vi "0Ludwieg_automation.vi"() -> ()   [LabVIEW 2025]
uses:
  State.ctl
  <vilib>/DAQmx/write.llb/DAQmx Write (Digital Bool 1Line 1Point).vi
  <vilib>/DAQmx/read.llb/DAQmx Read (Analog 2D DBL NChan NSamp).vi
  <vilib>/Analysis/baseanly.llb/Mean (DBL).vi
  <vilib>/DAQmx/write.llb/DAQmx Write (Analog 2D DBL NChan NSamp).vi
  <vilib>/DAQmx/write.llb/DAQmx Write (Digital 1D U32 1Chan NSamp).vi
  <vilib>/DAQmx/write.llb/DAQmx Write (Analog 1D DBL NChan 1Samp).vi
  <vilib>/DAQmx/create/channels.llb/DAQmx Create Channel (DO-Digital Output).vi
  <vilib>/DAQmx/create/channels.llb/DAQmx Create Channel (AI-Voltage-Basic).vi
  <vilib>/DAQmx/configure/timing.llb/DAQmx Timing (Sample Clock).vi
  <vilib>/DAQmx/configure/trigger.llb/DAQmx Start Trigger (Digital Edge).vi
  <vilib>/DAQmx/create/channels.llb/DAQmx Create Channel (AO-Voltage-Basic).vi
  <vilib>/DAQmx/miscellaneous.llb/DAQmx Fill In Error Info.vi
  <vilib>/Analysis/NI_AALBase.lvlib
  <resource>/objmgr/daqmx.rc
panel:
  out "Write_OK":bool
  in  "Done?":bool
  in  "Write?":bool
  in  "Start_path":path=path "C:/Users/IITH/Desktop"
  out "Saved_file_path":path
  out "Last_run?":bool
  in  "Next_run?":bool
  out "Timing_OK":bool
  out "Timing_msg":string
  out "gate_start_ms":dbl
  in  "trigger_gap_ms":dbl=-1.0
  in  "Cam_gate_len_ms":dbl=40.0
  in  "pre_flow_ms":dbl=15.0
  in  "flow_lag_ms":dbl=30.0
  in  "valve_delay":dbl=100.0
  in  "Valve_pulse_ms":dbl=30.0
  out "Camera_delay":dbl=50.0
  in  "Camera_pulse_ms":dbl=50.0
  out "Pulse_length_ms":dbl=500.0
  in  "AI_Start_delay_ms":dbl=115.0
  in  "AI_Capture_ms":dbl=40.0
  out "Run_count":i32
  in  "N_runs":i32=1 min=1 max=10 step=1
  out "Iteration":i32
  out "Current_state":T1
  in  "AI_data_record_Ch":tag="Dev1/ai0:3"
  out "Actual_AI_Rate":dbl
  in  "Frequency (Hz)":dbl=300000.0 format="%0.2f"
  in  "Abort":bool
  in  "Force_stop":bool
  in  "Vac_pump_DO_Ch":tag="Dev1/port1/line1"
  in  "Fire_AO_Ch":tag="Dev1/ao0:1"
  in  "AI_input_config":i32(ring)=10106 items=["Default"=-1, "RSE"=10083, "NRSE"=10078, "Differential"=10106, "Pseudodifferential"=12529]
  in  "Global_driver_rate":dbl=1000.0 format="%0.2f"
  in  "Exhaust_SSR_Ch":tag="Dev2/ao1"
  in  "Inlet_SSR_Ch":tag="Dev2/ao0"
  out "Vac_Pump":bool
  out "Abort_state":bool
  out "P_vac_Pa":dbl
  out "P_driver_Pa":dbl
  out "Fill_cutoff_Pa":dbl format="%.4f"
  out "Vac_cutoff_Pa":dbl format="%.4f"
  in  "Driver_units":enum16{"psi", "bar", "kPa", "Pa"}(ring)=enum."bar"
  in  "Vacuum_units":enum16{"psi", "bar", "kPa", "Pa"}(ring)=enum."Pa"
  in  "P_driver_target":dbl=10.0
  in  "P_vac_target":dbl=6.0
  in  "Vac_pressure_Ch":tag="Dev2/ai0"
  in  "Driver_pressure_Ch":tag="Dev2/ai1"
  out "Driver_gauge_%":dbl(knob) scale=0.0..130.0
  out "Vac_gauge_%":dbl(knob)
  out "Sensor_fault":bool
  out "Control_pressures":dbl[][](graph)
  out "6374_data_output":dbl[][](graph)
  out "Trigger_pulse_waveform":dbl[][](graph)=[[0.0, 0.0, 0.0, 0.0, 0.0, 0.0, 0.0, 0.0, 0.0, 0.0, 0.0, 0.0, 0.0, 0.0, 0.0, 0.0, 0.0, 0.0, 0.0, 0.0, 0.0, 0.0, 0.0, 0.0, 0.0, 0.0, 0.0, 0.0, 0.0, 0.0, 0.0, 0.0, 0.0, 0.0, 0.0, 0.0, 0.0, 0.0, 0.0, 0.0, 0.0, 0.0, 0.0, 0.0, 0.0, 0.0, 0.0, 0.0, 0.0, 0.0, 0.0, 0.0, 0.0, 0.0, 0.0, 0.0, 0.0, 0.0, 0.0, 0.0, 0.0, 0.0, 0.0, 0.0, 0.0, 0.0, 0.0, 0.0, 0.0, 0.0, 0.0, 0.0, 0.0, 0.0, 0.0, 0.0, 0.0, 0.0, 0.0, 0.0, 0.0, 0.0, 0.0, 0.0, 0.0, 0.0, 0.0, 0.0, 0.0, 0.0, 0.0, 0.0, 0.0, 0.0, 0.0, 0.0, 0.0, 0.0, 0.0, 0.0, 4.9, 4.9, 4.9, 4.9, 4.9, 4.9, 4.9, 4.9, 4.9, 4.9, 4.9, 4.9, 4.9, 4.9, 4.9, 4.9, 4.9, 4.9, 4.9, 4.9, 4.9, 4.9, 4.9, 4.9, 4.9, 4.9, 4.9, 4.9, 4.9, 4.9, 4.9, 4.9, 4.9, 4.9, 4.9, 4.9, 4.9, 4.9, 4.9, 4.9, 4.9, 4.9, 4.9, 4.9, 4.9, 4.9, 4.9, 4.9, 4.9, 4.9, 0.0, 0.0, 0.0, 0.0, 0.0, 0.0, 0.0, 0.0, 0.0, 0.0, 0.0, 0.0, 0.0, 0.0, 0.0, 0.0, 0.0, 0.0, 0.0, 0.0, 0.0, 0.0, 0.0, 0.0, 0.0, 0.0, 0.0, 0.0, 0.0, 0.0, 0.0, 0.0, 0.0, 0.0, 0.0, 0.0, 0.0, 0.0, 0.0, 0.0, 0.0, 0.0, 0.0, 0.0, 0.0, 0.0, 0.0, 0.0, 0.0, 0.0, 0.0, 0.0, 0.0, 0.0, 0.0, 0.0, 0.0, 0.0, 0.0, 0.0, 0.0, 0.0, 0.0, 0.0, 0.0, 0.0, 0.0, 0.0, 0.0, 0.0, 0.0, 0.0, 0.0, 0.0, 0.0, 0.0, 0.0, 0.0, 0.0, 0.0, 0.0, 0.0, 0.0, 0.0, 0.0, 0.0, 0.0, 0.0, 0.0, 0.0, 0.0, 0.0, 0.0, 0.0, 0.0, 0.0, 0.0, 0.0, 0.0, 0.0, 0.0, 0.0, 0.0, 0.0, 0.0, 0.0, 0.0, 0.0, 0.0, 0.0, 0.0, 0.0, 0.0, 0.0, 0.0, 0.0, 0.0, 0.0, 0.0, 0.0, 0.0, 0.0, 0.0, 0.0, 0.0, 0.0, 0.0, 0.0, 0.0, 0.0, 0.0, 0.0, 0.0, 0.0, 0.0, 0.0, 0.0, 0.0, 0.0, 0.0, 0.0, 0.0, 0.0, 0.0, 0.0, 0.0, 0.0, 0.0, 0.0, 0.0, 0.0, 0.0, 0.0, 0.0, 0.0, 0.0, 0.0, 0.0, 0.0, 0.0, 0.0, 0.0, 0.0, 0.0, 0.0, 0.0, 0.0, 0.0, 0.0, 0.0, 0.0, 0.0, 0.0, 0.0, 0.0, 0.0, 0.0, 0.0, 0.0, 0.0, 0.0, 0.0, 0.0, 0.0, 0.0, 0.0, 0.0, 0.0, 0.0, 0.0, 0.0, 0.0, 0.0, 0.0, 0.0, 0.0, 0.0, 0.0, 0.0, 0.0, 0.0, 0.0, 0.0, 0.0, 0.0, 0.0, 0.0, 0.0, 0.0, 0.0, 0.0, 0.0, 0.0, 0.0, 0.0, 0.0, 0.0, 0.0, 0.0, 0.0, 0.0, 0.0, 0.0, 0.0, 0.0, 0.0, 0.0, 0.0, 0.0, 0.0, 0.0, 0.0, 0.0, 0.0, 0.0, 0.0, 0.0, 0.0, 0.0, 0.0, 0.0, 0.0, 0.0, 0.0, 0.0, 0.0, 0.0, 0.0, 0.0, 0.0, 0.0, 0.0, 0.0, 0.0, 0.0, 0.0, 0.0, 0.0, 0.0, 0.0, 0.0, 0.0, 0.0, 0.0, 0.0, 0.0, 0.0, 0.0, 0.0, 0.0, 0.0, 0.0, 0.0, 0.0, 0.0, 0.0, 0.0, 0.0, 0.0, 0.0, 0.0, 0.0, 0.0, 0.0, 0.0, 0.0, 0.0, 0.0, 0.0, 0.0, 0.0, 0.0, 0.0, 0.0, 0.0, 0.0, 0.0, 0.0, 0.0, 0.0, 0.0, 0.0, 0.0, 0.0, 0.0, 0.0, 0.0, 0.0, 0.0, 0.0, 0.0, 0.0, 0.0, 0.0, 0.0, 0.0, 0.0, 0.0, 0.0, 0.0, 0.0, 0.0, 0.0, 0.0, 0.0, 0.0, 0.0, 0.0, 0.0, 0.0, 0.0, 0.0, 0.0, 0.0, 0.0, 0.0, 0.0, 0.0, 0.0, 0.0, 0.0, 0.0, 0.0, 0.0, 0.0, 0.0, 0.0, 0.0, 0.0, 0.0, 0.0, 0.0, 0.0, 0.0, 0.0, 0.0, 0.0, 0.0, 0.0, 0.0, 0.0, 0.0, 0.0, 0.0, 0.0, 0.0, 0.0, 0.0, 0.0, 0.0, 0.0, 0.0, 0.0, 0.0, 0.0, 0.0, 0.0, 0.0, 0.0, 0.0, 0.0, 0.0, 0.0, 0.0, 0.0, 0.0, 0.0, 0.0, 0.0, 0.0, 0.0, 0.0, 0.0, 0.0, 0.0, 0.0, 0.0, 0.0, 0.0, 0.0, 0.0, 0.0, 0.0, 0.0, 0.0, 0.0, 0.0, 0.0, 0.0, 0.0, 0.0, 0.0, 0.0, 0.0, 0.0, 0.0, 0.0, 0.0, 0.0, 0.0, 0.0, 0.0, 0.0, 0.0, 0.0, 0.0, 0.0, 0.0, 0.0, 0.0, 0.0, 0.0, 0.0, 0.0, 0.0, 0.0, 0.0, 0.0, 0.0, 0.0, 0.0, 0.0, 0.0, 0.0, 0.0, 0.0, 0.0, 0.0, 0.0, 0.0, 0.0, 0.0, 0.0, 0.0, 0.0, 0.0, 0.0, 0.0, 0.0, 0.0, 0.0, 0.0, 0.0, 0.0, 0.0, 0.0, 0.0, 0.0, 0.0, 0.0, 0.0, 0.0, 0.0, 0.0, 0.0, 0.0, 0.0, 0.0, 0.0, 0.0, 0.0, 0.0, 0.0, 0.0, 0.0, 0.0, 0.0, 0.0, 0.0, 0.0, 0.0, 0.0, 0.0, 0.0, 0.0, 0.0, 0.0, 0.0, 0.0, 0.0, 0.0, 0.0, 0.0, 0.0, 0.0, 0.0, 0.0, 0.0, 0.0, 0.0, 0.0, 0.0, 0.0, 0.0, 0.0, 0.0, 0.0, 0.0, 0.0, 0.0, 0.0, 0.0, 0.0, 0.0, 0.0, 0.0, 0.0, 0.0, 0.0, 0.0, 0.0, 0.0, 0.0, 0.0, 0.0, 0.0, 0.0, 0.0, 0.0, 0.0, 0.0, 0.0, 0.0, 0.0, 0.0, 0.0, 0.0, 0.0, 0.0, 0.0, 0.0, 0.0, 0.0, 0.0, 0.0, 0.0, 0.0, 0.0, 0.0, 0.0, 0.0, 0.0, 0.0, 0.0, 0.0, 0.0, 0.0, 0.0, 0.0, 0.0, 0.0, 0.0, 0.0, 0.0, 0.0, 0.0, 0.0, 0.0, 0.0, 0.0, 0.0, 0.0, 0.0, 0.0, 0.0, 0.0, 0.0, 0.0, 0.0, 0.0, 0.0, 0.0, 0.0, 0.0, 0.0, 0.0, 0.0, 0.0, 0.0, 0.0, 0.0, 0.0, 0.0, 0.0, 0.0, 0.0, 0.0, 0.0, 0.0, 0.0, 0.0, 0.0, 0.0, 0.0, 0.0, 0.0, 0.0, 0.0, 0.0, 0.0, 0.0, 0.0, 0.0, 0.0, 0.0, 0.0, 0.0, 0.0, 0.0, 0.0, 0.0, 0.0, 0.0, 0.0, 0.0, 0.0, 0.0, 0.0, 0.0, 0.0, 0.0, 0.0, 0.0, 0.0, 0.0, 0.0, 0.0, 0.0, 0.0, 0.0, 0.0, 0.0, 0.0, 0.0, 0.0, 0.0, 0.0, 0.0, 0.0, 0.0, 0.0, 0.0, 0.0, 0.0, 0.0, 0.0, 0.0, 0.0, 0.0, 0.0, 0.0, 0.0, 0.0, 0.0, 0.0, 0.0, 0.0, 0.0, 0.0, 0.0, 0.0, 0.0, 0.0, 0.0, 0.0, 0.0, 0.0, 0.0, 0.0, 0.0, 0.0, 0.0, 0.0, 0.0, 0.0, 0.0, 0.0, 0.0, 0.0, 0.0, 0.0, 0.0, 0.0, 0.0, 0.0, 0.0, 0.0, 0.0, 0.0, 0.0, 0.0, 0.0, 0.0, 0.0, 0.0, 0.0, 0.0, 0.0, 0.0, 0.0, 0.0, 0.0, 0.0, 0.0, 0.0, 0.0, 0.0, 0.0, 0.0, 0.0, 0.0, 0.0, 0.0, 0.0, 0.0, 0.0, 0.0, 0.0, 0.0, 0.0, 0.0, 0.0, 0.0, 0.0, 0.0, 0.0, 0.0, 0.0, 0.0, 0.0, 0.0, 0.0, 0.0, 0.0, 0.0, 0.0, 0.0, 0.0, 0.0, 0.0, 0.0, 0.0, 0.0, 0.0, 0.0, 0.0, 0.0, 0.0, 0.0, 0.0, 0.0, 0.0, 0.0, 0.0, 0.0, 0.0, 0.0, 0.0, 0.0, 0.0, 0.0, 0.0, 0.0, 0.0, 0.0, 0.0, 0.0, 0.0, 0.0, 0.0, 0.0, 0.0, 0.0, 0.0, 0.0, 0.0, 0.0, 0.0, 0.0, 0.0, 0.0, 0.0, 0.0, 0.0, 0.0, 0.0, 0.0, 0.0, 0.0, 0.0, 0.0, 0.0, 0.0, 0.0, 0.0, 0.0, 0.0, 0.0, 0.0, 0.0, 0.0, 0.0, 0.0, 0.0, 0.0, 0.0, 0.0, 0.0, 0.0, 0.0, 0.0, 0.0, 0.0, 0.0, 0.0, 0.0, 0.0, 0.0, 0.0, 0.0, 0.0, 0.0, 0.0, 0.0, 0.0, 0.0, 0.0, 0.0, 0.0, 0.0], [0.0, 0.0, 0.0, 0.0, 0.0, 0.0, 0.0, 0.0, 0.0, 0.0, 0.0, 0.0, 0.0, 0.0, 0.0, 0.0, 0.0, 0.0, 0.0, 0.0, 0.0, 0.0, 0.0, 0.0, 0.0, 0.0, 0.0, 0.0, 0.0, 0.0, 0.0, 0.0, 0.0, 0.0, 0.0, 0.0, 0.0, 0.0, 0.0, 0.0, 0.0, 0.0, 0.0, 0.0, 0.0, 0.0, 0.0, 0.0, 0.0, 0.0, 0.0, 0.0, 0.0, 0.0, 0.0, 0.0, 0.0, 0.0, 0.0, 0.0, 0.0, 0.0, 0.0, 0.0, 0.0, 0.0, 0.0, 0.0, 0.0, 0.0, 0.0, 0.0, 0.0, 0.0, 0.0, 0.0, 0.0, 0.0, 0.0, 0.0, 0.0, 0.0, 0.0, 0.0, 0.0, 0.0, 0.0, 0.0, 0.0, 0.0, 0.0, 0.0, 0.0, 0.0, 0.0, 0.0, 0.0, 0.0, 0.0, 0.0, 0.0, 0.0, 0.0, 0.0, 0.0, 0.0, 0.0, 0.0, 0.0, 0.0, 0.0, 0.0, 0.0, 0.0, 0.0, 0.0, 0.0, 0.0, 0.0, 0.0, 0.0, 0.0, 0.0, 0.0, 0.0, 0.0, 0.0, 0.0, 0.0, 0.0, 0.0, 0.0, 0.0, 0.0, 0.0, 0.0, 0.0, 0.0, 0.0, 0.0, 0.0, 0.0, 0.0, 0.0, 0.0, 0.0, 0.0, 0.0, 0.0, 0.0, 0.0, 0.0, 0.0, 0.0, 0.0, 0.0, 0.0, 0.0, 0.0, 0.0, 0.0, 0.0, 0.0, 0.0, 0.0, 0.0, 0.0, 0.0, 0.0, 0.0, 0.0, 0.0, 0.0, 0.0, 0.0, 0.0, 0.0, 0.0, 0.0, 0.0, 0.0, 0.0, 0.0, 0.0, 0.0, 0.0, 0.0, 0.0, 0.0, 0.0, 0.0, 0.0, 0.0, 0.0, 0.0, 0.0, 0.0, 0.0, 0.0, 0.0, 4.9, 4.9, 4.9, 4.9, 4.9, 4.9, 4.9, 4.9, 4.9, 4.9, 4.9, 4.9, 4.9, 4.9, 4.9, 4.9, 4.9, 4.9, 4.9, 4.9, 4.9, 4.9, 4.9, 4.9, 4.9, 4.9, 4.9, 4.9, 4.9, 4.9, 4.9, 4.9, 4.9, 4.9, 4.9, 4.9, 4.9, 4.9, 4.9, 4.9, 4.9, 4.9, 4.9, 4.9, 4.9, 4.9, 4.9, 4.9, 4.9, 4.9, 4.9, 4.9, 4.9, 4.9, 4.9, 4.9, 4.9, 4.9, 4.9, 4.9, 4.9, 4.9, 4.9, 4.9, 4.9, 4.9, 4.9, 4.9, 4.9, 4.9, 4.9, 4.9, 4.9, 4.9, 4.9, 4.9, 4.9, 4.9, 4.9, 4.9, 4.9, 4.9, 4.9, 4.9, 4.9, 4.9, 4.9, 4.9, 4.9, 4.9, 4.9, 4.9, 4.9, 4.9, 4.9, 4.9, 4.9, 4.9, 4.9, 4.9, 0.0, 0.0, 0.0, 0.0, 0.0, 0.0, 0.0, 0.0, 0.0, 0.0, 0.0, 0.0, 0.0, 0.0, 0.0, 0.0, 0.0, 0.0, 0.0, 0.0, 0.0, 0.0, 0.0, 0.0, 0.0, 0.0, 0.0, 0.0, 0.0, 0.0, 0.0, 0.0, 0.0, 0.0, 0.0, 0.0, 0.0, 0.0, 0.0, 0.0, 0.0, 0.0, 0.0, 0.0, 0.0, 0.0, 0.0, 0.0, 0.0, 0.0, 0.0, 0.0, 0.0, 0.0, 0.0, 0.0, 0.0, 0.0, 0.0, 0.0, 0.0, 0.0, 0.0, 0.0, 0.0, 0.0, 0.0, 0.0, 0.0, 0.0, 0.0, 0.0, 0.0, 0.0, 0.0, 0.0, 0.0, 0.0, 0.0, 0.0, 0.0, 0.0, 0.0, 0.0, 0.0, 0.0, 0.0, 0.0, 0.0, 0.0, 0.0, 0.0, 0.0, 0.0, 0.0, 0.0, 0.0, 0.0, 0.0, 0.0, 0.0, 0.0, 0.0, 0.0, 0.0, 0.0, 0.0, 0.0, 0.0, 0.0, 0.0, 0.0, 0.0, 0.0, 0.0, 0.0, 0.0, 0.0, 0.0, 0.0, 0.0, 0.0, 0.0, 0.0, 0.0, 0.0, 0.0, 0.0, 0.0, 0.0, 0.0, 0.0, 0.0, 0.0, 0.0, 0.0, 0.0, 0.0, 0.0, 0.0, 0.0, 0.0, 0.0, 0.0, 0.0, 0.0, 0.0, 0.0, 0.0, 0.0, 0.0, 0.0, 0.0, 0.0, 0.0, 0.0, 0.0, 0.0, 0.0, 0.0, 0.0, 0.0, 0.0, 0.0, 0.0, 0.0, 0.0, 0.0, 0.0, 0.0, 0.0, 0.0, 0.0, 0.0, 0.0, 0.0, 0.0, 0.0, 0.0, 0.0, 0.0, 0.0, 0.0, 0.0, 0.0, 0.0, 0.0, 0.0, 0.0, 0.0, 0.0, 0.0, 0.0, 0.0, 0.0, 0.0, 0.0, 0.0, 0.0, 0.0, 0.0, 0.0, 0.0, 0.0, 0.0, 0.0, 0.0, 0.0, 0.0, 0.0, 0.0, 0.0, 0.0, 0.0, 0.0, 0.0, 0.0, 0.0, 0.0, 0.0, 0.0, 0.0, 0.0, 0.0, 0.0, 0.0, 0.0, 0.0, 0.0, 0.0, 0.0, 0.0, 0.0, 0.0, 0.0, 0.0, 0.0, 0.0, 0.0, 0.0, 0.0, 0.0, 0.0, 0.0, 0.0, 0.0, 0.0, 0.0, 0.0, 0.0, 0.0, 0.0, 0.0, 0.0, 0.0, 0.0, 0.0, 0.0, 0.0, 0.0, 0.0, 0.0, 0.0, 0.0, 0.0, 0.0, 0.0, 0.0, 0.0, 0.0, 0.0, 0.0, 0.0, 0.0, 0.0, 0.0, 0.0, 0.0, 0.0, 0.0, 0.0, 0.0, 0.0, 0.0, 0.0, 0.0, 0.0, 0.0, 0.0, 0.0, 0.0, 0.0, 0.0, 0.0, 0.0, 0.0, 0.0, 0.0, 0.0, 0.0, 0.0, 0.0, 0.0, 0.0, 0.0, 0.0, 0.0, 0.0, 0.0, 0.0, 0.0, 0.0, 0.0, 0.0, 0.0, 0.0, 0.0, 0.0, 0.0, 0.0, 0.0, 0.0, 0.0, 0.0, 0.0, 0.0, 0.0, 0.0, 0.0, 0.0, 0.0, 0.0, 0.0, 0.0, 0.0, 0.0, 0.0, 0.0, 0.0, 0.0, 0.0, 0.0, 0.0, 0.0, 0.0, 0.0, 0.0, 0.0, 0.0, 0.0, 0.0, 0.0, 0.0, 0.0, 0.0, 0.0, 0.0, 0.0, 0.0, 0.0, 0.0, 0.0, 0.0, 0.0, 0.0, 0.0, 0.0, 0.0, 0.0, 0.0, 0.0, 0.0, 0.0, 0.0, 0.0, 0.0, 0.0, 0.0, 0.0, 0.0, 0.0, 0.0, 0.0, 0.0, 0.0, 0.0, 0.0, 0.0, 0.0, 0.0, 0.0, 0.0, 0.0, 0.0, 0.0, 0.0, 0.0, 0.0, 0.0, 0.0, 0.0, 0.0, 0.0, 0.0, 0.0, 0.0, 0.0, 0.0, 0.0, 0.0, 0.0, 0.0, 0.0, 0.0, 0.0, 0.0, 0.0, 0.0, 0.0, 0.0, 0.0, 0.0, 0.0, 0.0, 0.0, 0.0, 0.0, 0.0, 0.0, 0.0, 0.0, 0.0, 0.0, 0.0, 0.0, 0.0, 0.0, 0.0, 0.0, 0.0, 0.0, 0.0, 0.0, 0.0, 0.0, 0.0, 0.0, 0.0, 0.0, 0.0, 0.0, 0.0, 0.0, 0.0, 0.0, 0.0, 0.0, 0.0, 0.0, 0.0, 0.0, 0.0, 0.0, 0.0, 0.0, 0.0, 0.0, 0.0, 0.0, 0.0, 0.0, 0.0, 0.0, 0.0, 0.0, 0.0, 0.0, 0.0, 0.0, 0.0, 0.0, 0.0, 0.0, 0.0, 0.0, 0.0, 0.0, 0.0, 0.0, 0.0, 0.0, 0.0, 0.0, 0.0, 0.0, 0.0, 0.0, 0.0, 0.0, 0.0, 0.0, 0.0, 0.0, 0.0, 0.0, 0.0, 0.0, 0.0, 0.0, 0.0, 0.0, 0.0, 0.0, 0.0, 0.0, 0.0, 0.0, 0.0, 0.0, 0.0, 0.0, 0.0, 0.0, 0.0, 0.0, 0.0, 0.0, 0.0, 0.0, 0.0, 0.0, 0.0, 0.0, 0.0, 0.0, 0.0, 0.0, 0.0, 0.0, 0.0, 0.0, 0.0, 0.0, 0.0, 0.0, 0.0, 0.0, 0.0, 0.0, 0.0, 0.0, 0.0, 0.0, 0.0, 0.0, 0.0, 0.0, 0.0, 0.0, 0.0, 0.0, 0.0, 0.0, 0.0, 0.0, 0.0, 0.0, 0.0, 0.0, 0.0, 0.0, 0.0, 0.0, 0.0, 0.0, 0.0, 0.0, 0.0, 0.0, 0.0, 0.0, 0.0, 0.0, 0.0, 0.0, 0.0, 0.0, 0.0, 0.0, 0.0, 0.0, 0.0, 0.0, 0.0, 0.0, 0.0, 0.0, 0.0, 0.0, 0.0, 0.0, 0.0, 0.0, 0.0, 0.0, 0.0, 0.0, 0.0, 0.0, 0.0, 0.0, 0.0, 0.0, 0.0, 0.0, 0.0, 0.0, 0.0, 0.0, 0.0, 0.0, 0.0, 0.0, 0.0, 0.0, 0.0, 0.0, 0.0, 0.0, 0.0, 0.0, 0.0, 0.0, 0.0, 0.0, 0.0, 0.0, 0.0, 0.0, 0.0, 0.0, 0.0, 0.0, 0.0, 0.0, 0.0, 0.0, 0.0, 0.0, 0.0, 0.0, 0.0, 0.0, 0.0, 0.0, 0.0, 0.0, 0.0, 0.0, 0.0, 0.0, 0.0, 0.0, 0.0, 0.0, 0.0, 0.0, 0.0, 0.0, 0.0, 0.0, 0.0, 0.0, 0.0, 0.0, 0.0, 0.0, 0.0, 0.0, 0.0, 0.0, 0.0, 0.0, 0.0, 0.0, 0.0, 0.0, 0.0, 0.0, 0.0, 0.0, 0.0, 0.0, 0.0, 0.0, 0.0, 0.0, 0.0, 0.0, 0.0]]
  out "Settling_chamber_pressure":dbl[](graph)
  # "Ludwieg Control Panel"
  # "Designed, Developed and Deployed by M. Raj Kiran Reddy"
  # "Only press next run after \nentering complete state"
  # "Dont touch - Unless you know what you are doing"
  # "PCIe_6374"
  # "USB_6003"
  # "USB_6003"
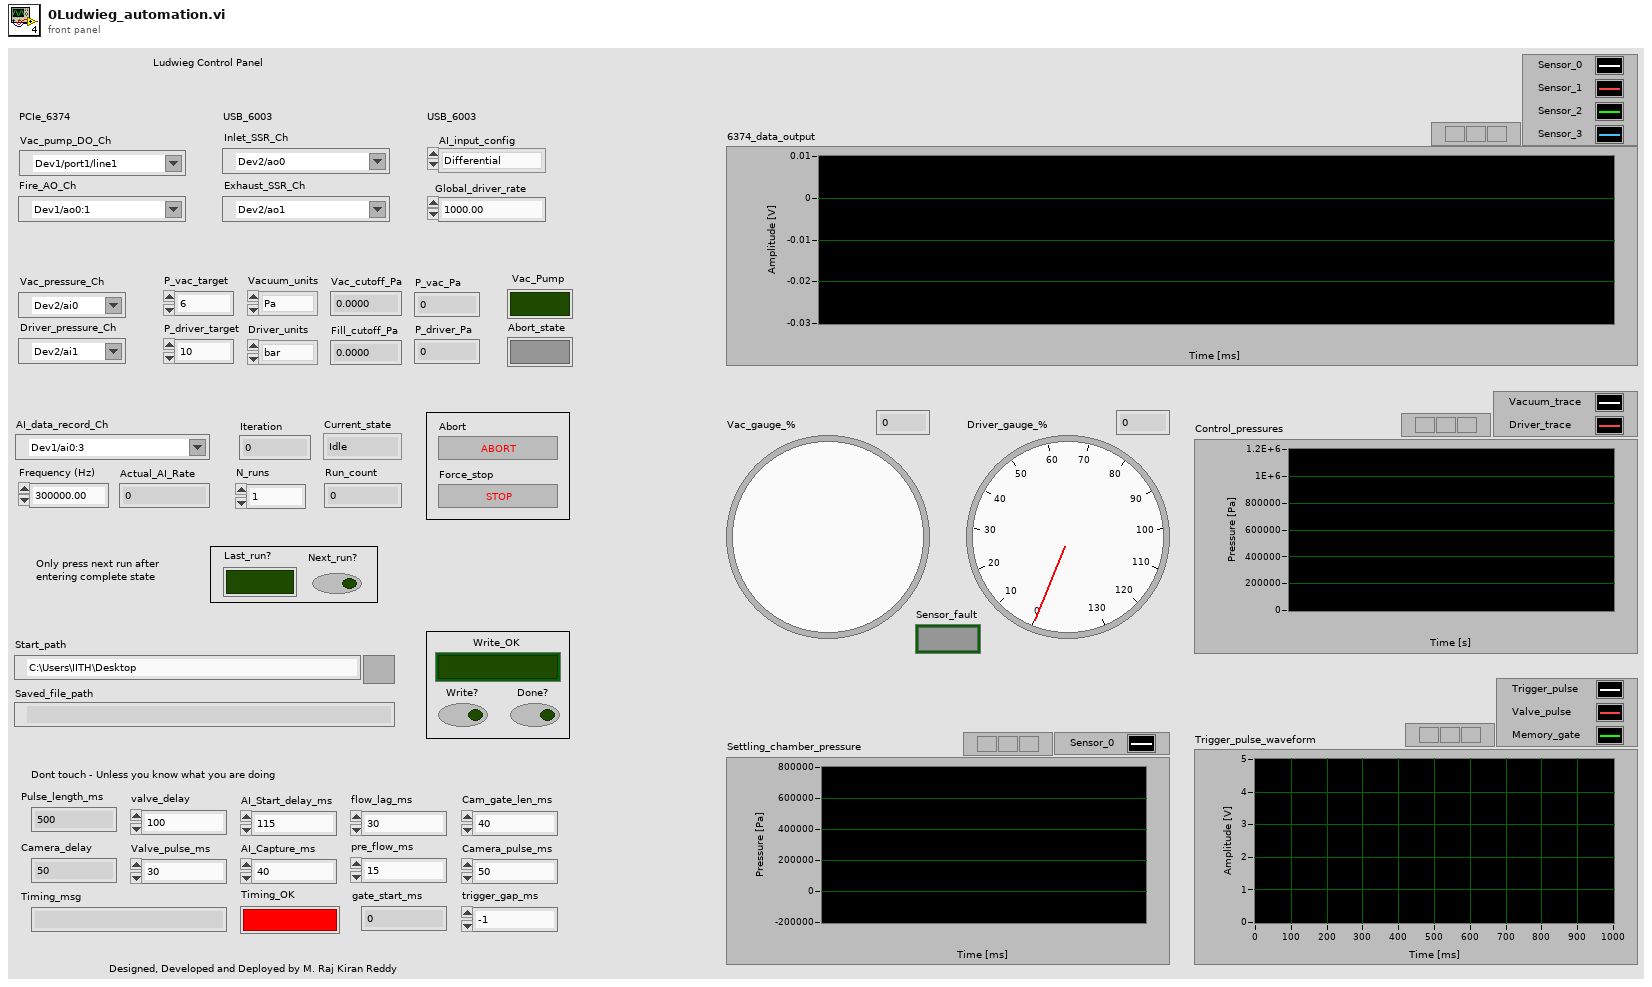
[diagram p1: front panel]
types:
  T1 = typedef "State.ctl" = enum16{"Idle", "WaitVac", "FillCoarse", "FillFine", "Hold", "Ready", "Firing", "Logging", "Complete", "Abort"}
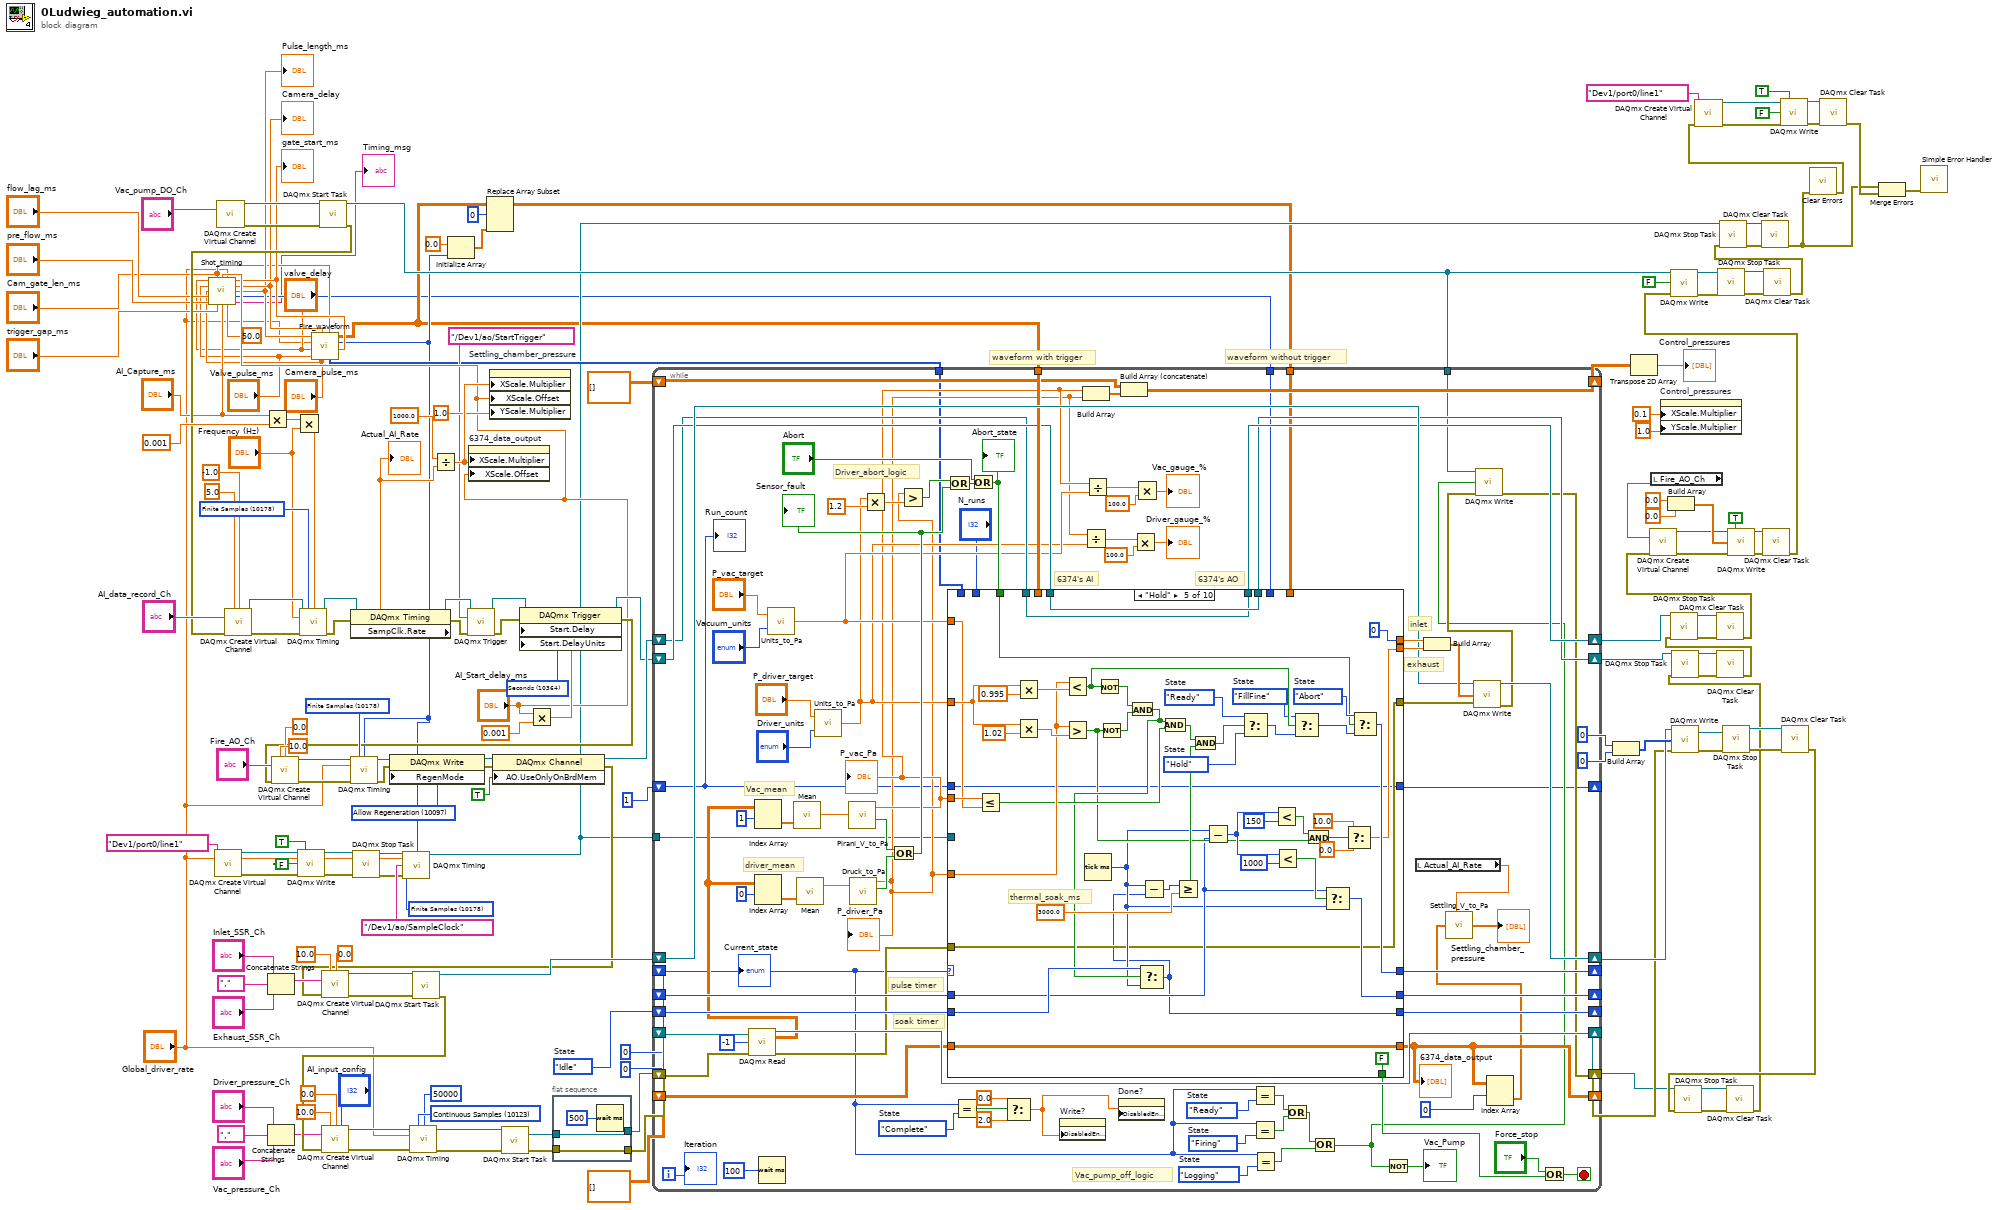
[diagram p0: block diagram]
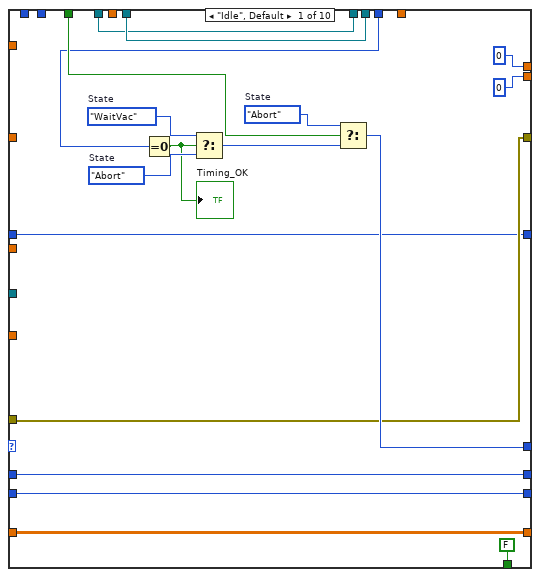
[diagram p2: hidden frame]
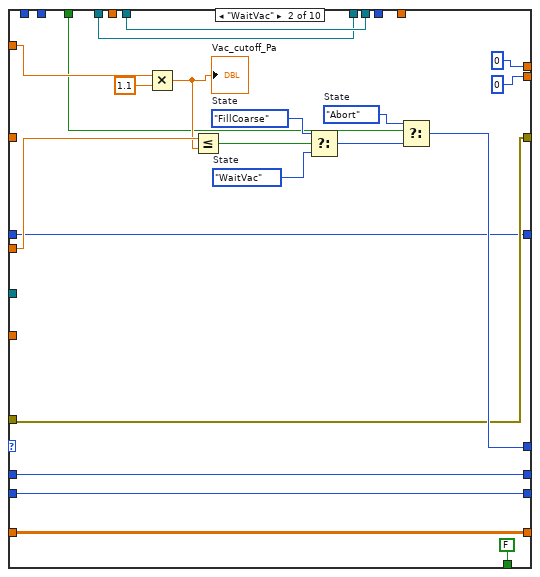
[diagram p3: hidden frame]
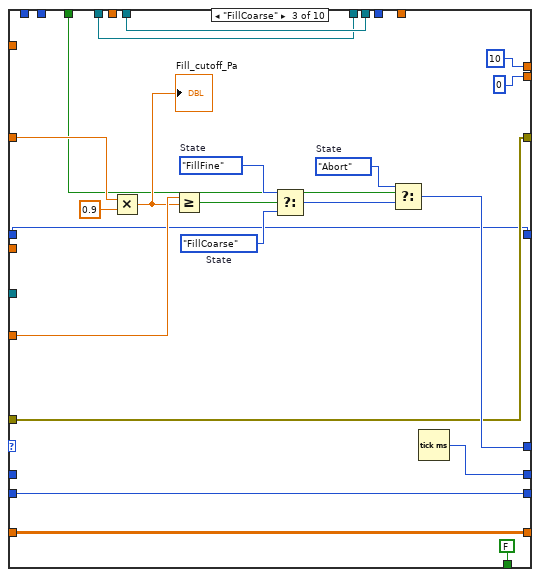
[diagram p4: hidden frame]
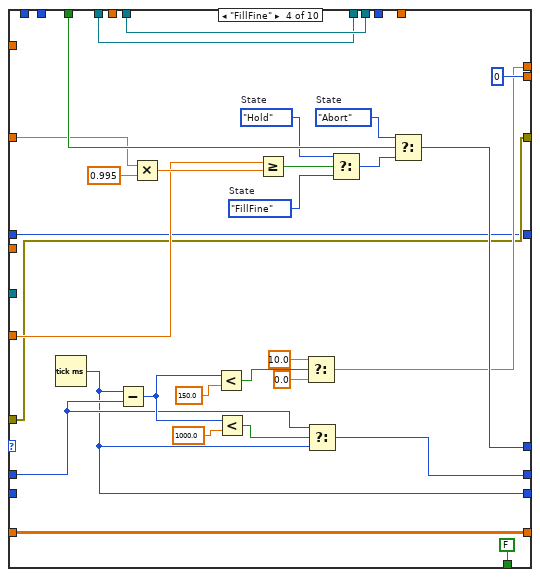
[diagram p5: hidden frame]
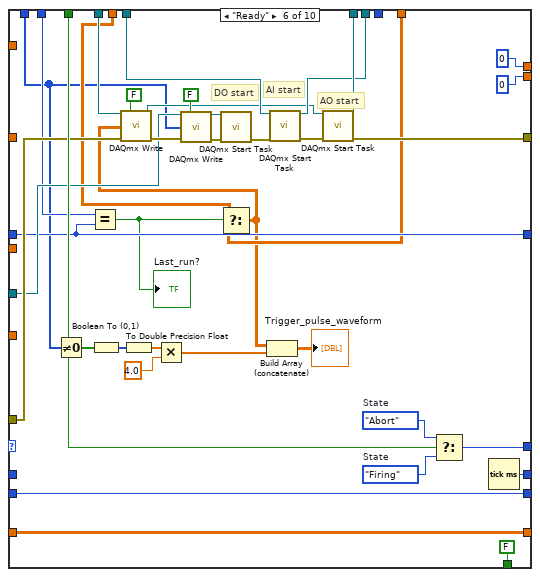
[diagram p6: hidden frame]
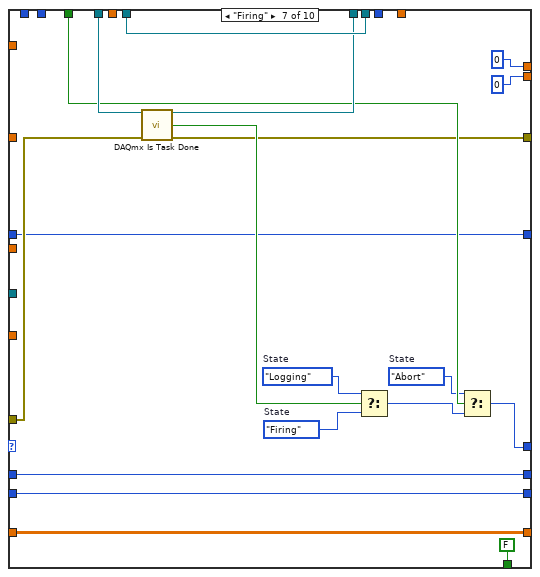
[diagram p7: hidden frame]
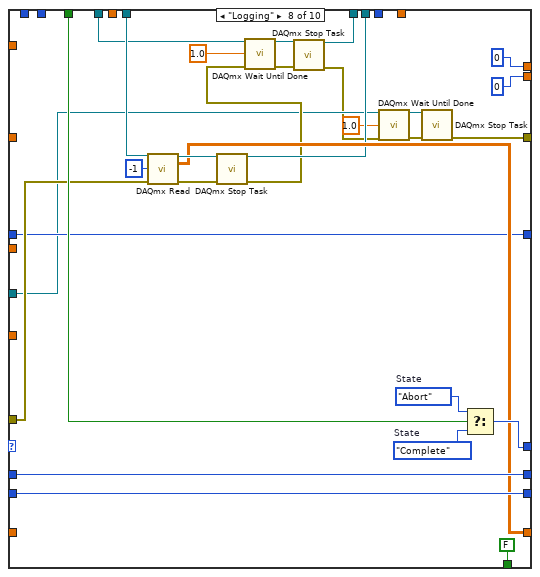
[diagram p8: hidden frame]
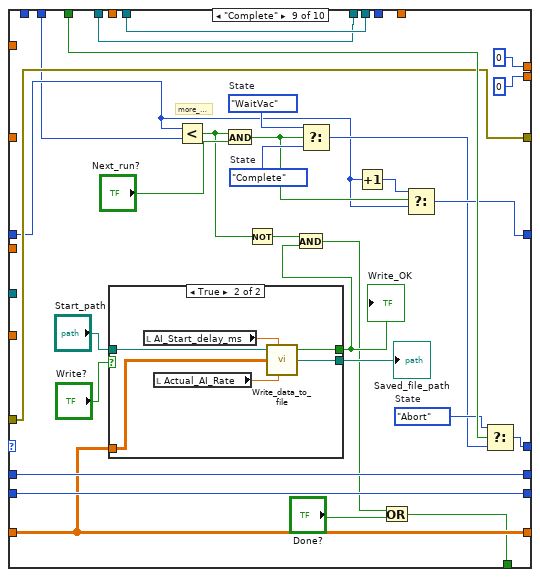
[diagram p9: hidden frame]
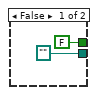
[diagram p10: hidden frame]
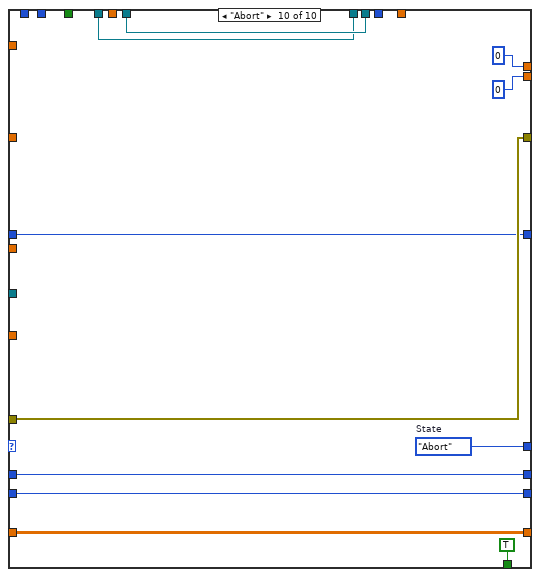
[diagram p11: hidden frame]
diagram:
  w29 = 10178 items=["Finite Samples"=10178, "Continuous Samples"=10123, "Hardware Timed Single Point"=12522] ("sample mode")
  w103 = 10364 items=["Sample Clock Periods"=10286, "Seconds"=10364, "Ticks"=10304] ("Start.DelayUnits")
  w110 = 10178 items=["Finite Samples"=10178, "Continuous Samples"=10123, "Hardware Timed Single Point"=12522] ("sample mode")
  w120 = 10178 items=["Finite Samples"=10178, "Continuous Samples"=10123, "Hardware Timed Single Point"=12522] ("sample mode")
  w123 = 10097 items=["Allow Regeneration"=10097, "Do Not Allow Regeneration"=10158] ("RegenMode")
  w160 = 10123 items=["Finite Samples"=10178, "Continuous Samples"=10123, "Hardware Timed Single Point"=12522] ("sample mode")
  w168 = State."Idle"  # State
  # "waveform without trigger"
  # "waveform with trigger"
  n1 = call "Shot_timing.vi"("valve_delay"="valve_delay", "gate_len_ms"="Cam_gate_len_ms", "start_delay_ms"="AI_Start_delay_ms", "rate"="Global_driver_rate", "valve_pulse_ms"="Valve_pulse_ms", "camera_pulse_ms"="Camera_pulse_ms", "flow_lag_ms"="flow_lag_ms", "pre_flow_ms"="pre_flow_ms", "trigger_gap_ms"="trigger_gap_ms", "capture_time_ms"="AI_Capture_ms", "tail_ms"=50.0) -> ("gate_start_ms"=w44:dbl, "camera_delay"=w43:dbl, "pulse_length_ms"=w42:dbl, "fail_code"=w2:i32, "Timing_msg"=→"Timing_msg":string)
  "Pulse_length_ms" <- w42
  "Camera_delay" <- w43
  "gate_start_ms" <- w44
  n2 = call-poly <vilib>:"DAQmx Create Virtual Channel.vi"("lines"=tag "Dev1/port0/line1") -> ("task out"=w36:refnum<k21>, "error out"=w35:errorcluster)  [unwired: 13 in]
  n3 = call-poly <vilib>:"DAQmx Create Virtual Channel.vi"("lines"="Vac_pump_DO_Ch") -> ("task out"=w74:refnum<k21>, "error out"=w73:errorcluster)  [unwired: 13 in]
  n4 = Multiply(x="AI_Capture_ms", y=0.001) -> (x*y=w104:dbl)
  n5 = Concatenate Strings("Inlet_SSR_Ch", tag "," ("string"), "Exhaust_SSR_Ch") -> (w154:string)
  n6 = Concatenate Strings("Driver_pressure_Ch", tag "," ("string"), "Vac_pressure_Ch") -> (w143:string)
  n7 = Multiply(x=w104, y="Frequency (Hz)") -> (x*y=w109:dbl)
  n8 = call-poly <vilib>:"DAQmx Write.vi"("task/channels in"=w36, "auto start"=TRUE, "data"=FALSE, "error in"=w35) -> ("task out"=w32:refnum<k21>, "error out"=w31:errorcluster)  [unwired: 9 in, 1 out]
  n9 = call "Fire_waveform.vi"("gate_start_ms"=w44, "gate_len_ms"="Cam_gate_len_ms", "camera_pulse_ms"="Camera_pulse_ms", "camera_delay"=w43, "valve_pulse_ms"="Valve_pulse_ms", "valve_delay"="valve_delay", "rate"="Global_driver_rate", "pulse_length_ms"=w42) -> ("N"=w7:i32, "waveform"=w6:dbl[][], "Gate"=w24:u32[])  [unwired: 1 in]
  n10 = call <vilib>:"DAQmx Start Task.vi"("task/channels in"=w74, "error in"=w73) -> ("task out"=w66:refnum<k21>, "error out"=w70:errorcluster)  [unwired: 12 in]
  n11 = call-poly <vilib>:"DAQmx Create Virtual Channel.vi"("maximum value"=5.0, "minimum value"=-1.0, "physical channels"="AI_data_record_Ch", "error in"=w70) -> ("task out"=w111:refnum<k21>, "error out"=w112:errorcluster)  [unwired: 10 in]
  n12 = call-poly <vilib>:"DAQmx Timing.vi"("task/channels in"=w111, "sample mode"=w110, "samples per channel"=w109, "rate"="Frequency (Hz)", "error in"=w112) -> ("task out"=w90:refnum<k21>, "error out"=w87:errorcluster)  [unwired: 9 in]
  n13 = property class="DAQmx Timing"(reference=w90, error in=w87) -> (reference out=w89:refnum<k21>, error out=w88:errorcluster, "SampClk.Rate"=w85:dbl)
  "Actual_AI_Rate" <- w85
  n14 = call <vilib>:"DAQmx Stop Task.vi"("task/channels in"=w32, "error in"=w31) -> ("task out"=w26:refnum<k21>, "error out"=w25:errorcluster)  [unwired: 12 in]
  n15 = call-poly <vilib>:"DAQmx Timing.vi"("task/channels in"=w26, "sample mode"=w29, "samples per channel"=w7, "rate"="Global_driver_rate", "source"=tag "/Dev1/ao/SampleClock", "error in"=w25) -> ("task out"=w14:refnum<k21>)  [unwired: 8 in, 1 out]
  n16 = Divide(x=1000.0, y=w85) -> (x/y=w82:dbl)
  n17 = Initialize Array(0.0 ("element"), w7) -> (w4:dbl[])
  n18 = call-poly <vilib>:"DAQmx Trigger.vi"("task/channels in"=w89, "source"=tag "/Dev1/ao/StartTrigger" ("Clock_ source"), "error in"=w88) -> ("task out"=w107:refnum<k21>, "error out"=w106:errorcluster)  [unwired: 11 in]
  n19 = property on="6374_data_output" class="WFGraph (strict)"("XScale.Multiplier"=w82, "XScale.Offset"="AI_Start_delay_ms") -> ()  [unwired: 2 in, 2 out]
  n20 = Replace Array Subset(array=w6, new element=w4, index (row)=0) -> (w3:dbl[][])  [unwired: 1 in]
  n21 = property on="Settling_chamber_pressure" class="WFGraph (strict)"("XScale.Multiplier"=w82, "XScale.Offset"="AI_Start_delay_ms", "YScale.Multiplier"=1.0 ("Y Scale.Offset and Multiplier:Multiplier")) -> ()  [unwired: 2 in, 2 out]
  n22 = Multiply(x="AI_Start_delay_ms", y=0.001) -> (x*y=w84:dbl)
  n23 = property class="DAQmx Trigger"(reference=w107, error in=w106, "Start.Delay"=w84, "Start.DelayUnits"=w103) -> (reference out=w101:refnum<k21>, error out=w93:errorcluster)
  n24 = call-poly <vilib>:"DAQmx Create Virtual Channel.vi"("maximum value"=10.0, "minimum value"=0.0, "physical channels"="Fire_AO_Ch", "error in"=w93) -> ("task out"=w119:refnum<k21>, "error out"=w116:errorcluster)  [unwired: 10 in]
  n25 = call-poly <vilib>:"DAQmx Timing.vi"("task/channels in"=w119, "sample mode"=w120, "samples per channel"=w7, "rate"="Global_driver_rate", "error in"=w116) -> ("task out"=w118:refnum<k21>, "error out"=w115:errorcluster)  [unwired: 9 in]
  n26 = property class="DAQmx Write"(reference=w118, error in=w115, "RegenMode"=w123) -> (reference out=w117:refnum<k21>, error out=w114:errorcluster)
  n27 = property class="DAQmx Channel"(reference=w117, error in=w114, "AO.UseOnlyOnBrdMem"=TRUE) -> (reference out=w113:refnum<k21>, error out=w92:errorcluster)
  n28 = call-poly <vilib>:"DAQmx Create Virtual Channel.vi"("maximum value"=10.0, "minimum value"=0.0, "physical channels"=w154, "error in"=w92) -> ("task out"=w150:refnum<k21>, "error out"=w151:errorcluster)  [unwired: 10 in]
  n29 = call <vilib>:"DAQmx Start Task.vi"("task/channels in"=w150, "error in"=w151) -> ("task out"=w149:refnum<k21>, "error out"=w148:errorcluster)  [unwired: 12 in]
  n30 = call-poly <vilib>:"DAQmx Create Virtual Channel.vi"("maximum value"=10.0, "minimum value"=0.0, "input terminal configuration"="AI_input_config", "physical channels"=w143, "error in"=w148) -> ("task out"=w162:refnum<k21>, "error out"=w158:errorcluster)  [unwired: 9 in]
  n31 = call-poly <vilib>:"DAQmx Timing.vi"("task/channels in"=w162, "sample mode"=w160, "samples per channel"=50000, "rate"="Global_driver_rate", "error in"=w158) -> ("task out"=w142:refnum<k21>, "error out"=w141:errorcluster)  [unwired: 9 in]
  n32 = call <vilib>:"DAQmx Start Task.vi"("task/channels in"=w142, "error in"=w141) -> ("task out"=w145:refnum<k21>, "error out"=w147:errorcluster)  [unwired: 12 in]
  n33 = flat-sequence {
    tunnel: w147 -> [w170]
    tunnel: [w170] -> w146
    tunnel: w145 -> [w169]
    tunnel: [w169] -> w144
    frame #0 {
      n34 = Wait (ms)(milliseconds to wait=u32 500) -> ()  [unwired: 1 out]
    }
  }
  n35 = while {
    shift-right: [w261] -> _
    shift-left: w168 -> [w203]
    shift-right: [w196] -> w132
    shift-left: w146 -> [w250]
    shift-right: [w260] -> w128
    shift-left: w144 -> [w251]
    shift-right: [w232] -> _
    shift-left: 0 -> [w233]
    shift-right: [w244] -> w137
    shift-left: w149 -> [w229]
    shift-right: [w230] -> _
    shift-left: 0 -> [w231]
    shift-right: [w225] -> w96
    shift-left: w101 -> [w227]
    shift-right: [w226] -> w54
    shift-left: w113 -> [w224]
    tunnel: w6 -> [w228]
    shift-right: [w212] -> _
    shift-left: dbl[][] [] -> [w221]
    shift-right: [w208] -> w79
    shift-left: dbl[][] [] -> [w209]
    tunnel: w66 -> [w204]
    shift-right: [w178] -> _
    shift-left: 1 -> [w177]
    tunnel: w24 -> [w176]
    tunnel: w14 -> [w175]
    tunnel: w3 -> [w173]
    tunnel: w2 -> [w172]
    i -> [w249]
    stop <- w214 stop-if-true
    w205 = State."Logging"  # State
    w206 = State."Firing"  # State
    w207 = State."Ready"  # State
    w220 = State."Complete"  # State
    # "Vac_pump_off_logic"
    # "6374's AO"
    # "6374's AI"
    # "soak timer"
    # "pulse timer"
    # "Driver_abort_logic"
    # "exhaust"
    # "inlet"
    # "Vac_mean"
    # "driver_mean"
    n36 = call-poly <vilib>:"DAQmx Read.vi"("task/channels in"=w251, "number of samples per channel"=-1, "error in"=w250) -> ("task out"=w260:refnum<k21>, "data"=w211:dbl[][], "error out"=w223:errorcluster)  [unwired: 10 in]
    n37 = Index Array(array=w211, index (row)=1) -> (element=w253:dbl[])  [unwired: 1 in]
    n38 = Index Array(array=w211, index (row)=0) -> (element=w254:dbl[])  [unwired: 1 in]
    n39 = Wait (ms)(milliseconds to wait=u32 100) -> ()  [unwired: 1 out]
    n40 = call "Units_to_Pa.vi"("Units"="Vacuum_units", "Value"="P_vac_target") -> ("P_Pa"=w184:dbl)
    n41 = call-poly <vilib>:"Mean.vi"("X"=w253) -> ("mean"=w182:dbl)  [unwired: 1 out]
    n42 = call-poly <vilib>:"Mean.vi"("X"=w254) -> ("mean"=w257:dbl)  [unwired: 1 out]
    n43 = call "Units_to_Pa.vi"("Units"="Driver_units", "Value"="P_driver_target") -> ("P_Pa"=w183:dbl)
    n44 = call "Pirani_V_to_Pa.vi"("V_in"=w182) -> ("P_Pa"=w180:dbl, "Sensor_fault"=w181:bool)  [unwired: 2 out]
    "P_vac_Pa" <- w180
    n45 = call "Druck_to_Pa.vi"("V_in"=w257) -> ("Out_of_range"=w256:bool, "P_abs_Pa"=w179:dbl)  [unwired: 4 in, 1 out]
    "P_driver_Pa" <- w179
    n46 = Multiply(x=w183, y=1.2) -> (x*y=w239:dbl)
    n47 = Or(x=w181, y=w256) -> (x .or. y?=w237:bool)
    "Sensor_fault" <- w237
    n48 = Greater?(x=w179, y=w239) -> (0:w238:bool)
    n49 = Or(x=w238, y=w237) -> (x .or. y?=w236:bool)
    n50 = Equal?(x=w203, y=w220) -> (x = y?=w219:bool)
    n51 = Or(x="Abort", y=w236) -> (x .or. y?=w234:bool)
    "Abort_state" <- w234
    n52 = case shown="\"Hold\"" w203 {
      tunnel: [w272 w288 w309 w348 w386 w425 w442 w479 w505 w532] -> w261
      tunnel: w180 -> [_ w296 _ _ w389 _ _ _ _ _]
      tunnel: w179 -> [_ _ w317 w335 w392 _ _ _ _ _]
      tunnel: w184 -> [_ w298 _ _ w388 _ _ _ _ _]
      tunnel: w183 -> [_ _ w319 w337 w397 _ _ _ _ _]
      tunnel: [0 0 10 w341 0 0 0 0 0 0] -> w242
      tunnel: [0 0 0 0 w362 0 0 0 0 0] -> w241
      tunnel: w234 -> [w273 w289 w310 w347 w379 w426 w445 w478 w507 _]
      tunnel: w233 -> [w271 w287 _ w340 w360 _ w453 w482 w509 w529]
      tunnel: [w271 w287 w308 w339 w358 w424 w453 w482 w509 w529] -> w232
      tunnel: w231 -> [w270 w286 w307 _ w375 w434 w452 w481 w508 w528]
      tunnel: [w270 w286 w307 w323 w352 w434 w452 w481 w508 w528] -> w230
      tunnel: w224 -> [w268 w284 w305 w327 w356 w433 w450 w465 w512 w526]
      tunnel: w228 -> [_ _ _ _ _ w409 _ _ _ _]
      tunnel: w227 -> [w269 w285 w306 w328 w357 w431 w451 w477 w513 w527]
      tunnel: [w268 w284 w305 w327 w356 w429 w449 w463 w512 w526] -> w226
      tunnel: [w269 w285 w306 w328 w357 w428 w451 w468 w513 w527] -> w225
      tunnel: w223 -> [w267 w283 w304 w326 w355 w422 w441 w475 w502 w524]
      tunnel: [w267 w283 w304 w326 w355 w421 w440 w456 w502 w524] -> w222
      tunnel: w221 -> [w266 w282 w303 w325 w354 w420 w439 _ w503 w525]
      tunnel: [w266 w282 w303 w325 w354 w420 w439 w471 w503 w525] -> w212
      tunnel: [FALSE ("Done") FALSE ("Done") FALSE ("Done") FALSE ("Done") FALSE ("Done") FALSE ("Done") FALSE ("Done") FALSE ("Done") w500 TRUE ("Done")] -> w198
      tunnel: [w264 w280 w301 w322 w351 w411 w437 w469 w494 w522] -> w178
      tunnel: w177 -> [w264 w280 w301 w322 w351 w411 w437 w469 w486 w522]
      tunnel: w176 -> [_ _ _ _ _ w401 _ _ _ _]
      tunnel: w175 -> [_ _ _ _ _ w413 _ w458 _ _]
      tunnel: "N_runs" -> [_ _ _ _ _ w410 _ _ w485 _]
      tunnel: w173 -> [_ _ _ _ _ w408 _ _ _ _]
      tunnel: w172 -> [w263 _ _ _ _ _ _ _ _ _]
      frame "Idle", Default {
        w275 = State."Abort"  # State
        w278 = State."Abort"  # State
        w279 = State."WaitVac"  # State
        n53 = Equal To 0?(x=w263) -> (x = 0?=w262:bool)
        "Timing_OK" <- w262
        n54 = Select(t=w279, s=w262, f=w278) -> (s? t:f=w274:T1)
        n55 = Select(t=w275, s=w273, f=w274) -> (s? t:f=w272:T1)
      }
      frame "WaitVac" {
        w291 = State."Abort"  # State
        w293 = State."WaitVac"  # State
        w294 = State."FillCoarse"  # State
        n56 = Multiply(x=w298, y=1.1) -> (x*y=w292:dbl)
        "Vac_cutoff_Pa" <- w292
        n57 = Less Or Equal?(x=w296, y=w292) -> (x <= y?=w295:bool)
        n58 = Select(t=w294, s=w295, f=w293) -> (s? t:f=w290:T1)
        n59 = Select(t=w291, s=w289, f=w290) -> (s? t:f=w288:T1)
      }
      frame "FillCoarse" {
        w312 = State."Abort"  # State
        w314 = State."FillCoarse"  # State
        w315 = State."FillFine"  # State
        n60 = Multiply(x=w319, y=0.9) -> (x*y=w313:dbl)
        "Fill_cutoff_Pa" <- w313
        n61 = Greater Or Equal?(x=w317, y=w313) -> (x >= y?=w316:bool)
        n62 = Select(t=w315, s=w316, f=w314) -> (s? t:f=w311:T1)
        n63 = Select(t=w312, s=w310, f=w311) -> (s? t:f=w309:T1)
        n64 = Tick Count (ms)() -> (millisecond timer value=w308:u32)
      }
      frame "FillFine" {
        w331 = State."FillFine"  # State
        w332 = State."Hold"  # State
        w349 = State."Abort"  # State
        n65 = Tick Count (ms)() -> (millisecond timer value=w323:u32)
        n66 = Subtract(x=w323, y=w340) -> (x-y=w344:u32)
        n67 = Multiply(x=w337, y=0.995) -> (x*y=w336:dbl)
        n68 = Less?(x=w344, y=150.0) -> (x < y?=w330:bool)
        n69 = Less?(x=w344, y=1000.0) -> (x < y?=w329:bool)
        n70 = Greater Or Equal?(x=w335, y=w336) -> (x >= y?=w334:bool)
        n71 = Select(t=10.0, s=w330, f=0.0) -> (s? t:f=w341:dbl)
        n72 = Select(t=w340, s=w329, f=w323) -> (s? t:f=w339:u32)
        n73 = Select(t=w332, s=w334, f=w331) -> (s? t:f=w333:T1)
        n74 = Select(t=w349, s=w347, f=w333) -> (s? t:f=w348:T1)
      }
      frame "Hold" {
        w381 = State."FillFine"  # State
        w383 = State."Hold"  # State
        w384 = State."Ready"  # State
        w387 = State."Abort"  # State
        # "thermal_soak_ms"
        n75 = Less Or Equal?(x=w389, y=w388) -> (x <= y?=w385:bool)
        n76 = Multiply(x=w397, y=0.995) -> (x*y=w394:dbl)
        n77 = Multiply(x=w397, y=1.02) -> (x*y=w393:dbl)
        n78 = Less?(x=w392, y=w394) -> (x < y?=w382:bool)
        n79 = Greater?(x=w392, y=w393) -> (0:w367:bool)
        n80 = Tick Count (ms)() -> (millisecond timer value=w359:u32)
        n81 = Not(x=w382) -> (.not. x?=w391:bool)
        n82 = Not(x=w367) -> (.not. x?=w390:bool)
        n83 = And(x=w391, y=w390) -> (x .and. y?=w374:bool)
        n84 = Select(t=w375, s=w374, f=w359) -> (s? t:f=w352:u32)
        n85 = Subtract(x=w359, y=w352) -> (x-y=w377:u32)
        n86 = And(x=w374, y=w385) -> (x .and. y?=w372:bool)
        n87 = Greater Or Equal?(x=w377, y=3000.0 ("Thermal_soak_ms")) -> (x >= y?=w373:bool)
        n88 = And(x=w372, y=w373) -> (x .and. y?=w371:bool)
        n89 = Subtract(x=w359, y=w360) -> (x-y=w370:u32)
        n90 = Select(t=w384, s=w371, f=w383) -> (s? t:f=w380:T1)
        n91 = Less?(x=w370, y=u32 150) -> (x < y?=w366:bool)
        n92 = Less?(x=w370, y=u32 1000) -> (x < y?=w361:bool)
        n93 = Select(t=w381, s=w382, f=w380) -> (s? t:f=w378:T1)
        n94 = And(x=w366, y=w367) -> (x .and. y?=w365:bool)
        n95 = Select(t=w360, s=w361, f=w359) -> (s? t:f=w358:u32)
        n96 = Select(t=10.0, s=w365, f=0.0) -> (s? t:f=w362:dbl)
        n97 = Select(t=w387, s=w379, f=w378) -> (s? t:f=w386:T1)
      }
      frame "Ready" {
        w423 = State."Firing"  # State
        w427 = State."Abort"  # State
        # "DO start"
        # "AO start"
        # "AI start"
        n98 = Not Equal To 0?(x=w401) -> (x != 0?=w406:bool[])
        n99 = Equal?(x=w410, y=w411) -> (x = y?=w407:bool)
        "Last_run?" <- w407
        n100 = Boolean To (0,1)(Boolean=w406) -> (0, 1=w405:i16[])
        n101 = To Double Precision Float(number=w405) -> (double precision float=w404:dbl[])
        n102 = Multiply(x=w404, y=4.0) -> (x*y=w402:dbl[])
        n103 = Select(t=w409, s=w407, f=w408) -> (s? t:f=w400:dbl[][])
        n104 = call-poly <vilib>:"DAQmx Write.vi"("task/channels in"=w433, "auto start"=FALSE, "data"=w400, "error in"=w422) -> ("task out"=w412:refnum<k21>, "error out"=w415:errorcluster)  [unwired: 9 in, 1 out]
        n105 = call-poly <vilib>:"DAQmx Write.vi"("task/channels in"=w413, "auto start"=FALSE, "data"=w401, "error in"=w415) -> ("task out"=w418:refnum<k21>, "error out"=w417:errorcluster)  [unwired: 9 in, 1 out]
        n106 = call <vilib>:"DAQmx Start Task.vi"("task/channels in"=w418, "error in"=w417) -> ("error out"=w416:errorcluster)  [unwired: 12 in, 1 out]
        n107 = Build Array (concatenate)(w400, w402) -> (→"Trigger_pulse_waveform":dbl[][])
        n108 = call <vilib>:"DAQmx Start Task.vi"("task/channels in"=w431, "error in"=w416) -> ("task out"=w428:refnum<k21>, "error out"=w430:errorcluster)  [unwired: 12 in]
        n109 = call <vilib>:"DAQmx Start Task.vi"("task/channels in"=w412, "error in"=w430) -> ("task out"=w429:refnum<k21>, "error out"=w421:errorcluster)  [unwired: 12 in]
        n110 = Select(t=w427, s=w426, f=w423) -> (s? t:f=w425:T1)
        n111 = Tick Count (ms)() -> (millisecond timer value=w424:u32)
      }
      frame "Firing" {
        w444 = State."Abort"  # State
        w447 = State."Firing"  # State
        w448 = State."Logging"  # State
        n112 = call <vilib>:"DAQmx Is Task Done.vi"("task/channels in"=w450, "error in"=w441) -> ("task out"=w449:refnum<k21>, "task done?"=w446:bool, "error out"=w440:errorcluster)  [unwired: 11 in]
        n113 = Select(t=w448, s=w446, f=w447) -> (s? t:f=w443:T1)
        n114 = Select(t=w444, s=w445, f=w443) -> (s? t:f=w442:T1)
      }
      frame "Logging" {
        w472 = State."Complete"  # State
        w480 = State."Abort"  # State
        n115 = call-poly <vilib>:"DAQmx Read.vi"("task/channels in"=w477, "number of samples per channel"=-1, "error in"=w475) -> ("task out"=w474:refnum<k21>, "data"=w471:dbl[][], "error out"=w473:errorcluster)  [unwired: 10 in]
        n116 = call <vilib>:"DAQmx Stop Task.vi"("task/channels in"=w474, "error in"=w473) -> ("task out"=w468:refnum<k21>, "error out"=w467:errorcluster)  [unwired: 12 in]
        n117 = call <vilib>:"DAQmx Wait Until Done.vi"("task/channels in"=w465, "timeout (sec)"=1.0, "error in"=w467) -> ("task out"=w464:refnum<k21>, "error out"=w466:errorcluster)  [unwired: 11 in]
        n118 = call <vilib>:"DAQmx Stop Task.vi"("task/channels in"=w464, "error in"=w466) -> ("task out"=w463:refnum<k21>, "error out"=w457:errorcluster)  [unwired: 12 in]
        n119 = call <vilib>:"DAQmx Wait Until Done.vi"("task/channels in"=w458, "timeout (sec)"=1.0, "error in"=w457) -> ("task out"=w461:refnum<k21>, "error out"=w460:errorcluster)  [unwired: 11 in]
        n120 = call <vilib>:"DAQmx Stop Task.vi"("task/channels in"=w461, "error in"=w460) -> ("error out"=w456:errorcluster)  [unwired: 12 in, 1 out]
        n121 = Select(t=w480, s=w478, f=w472) -> (s? t:f=w479:T1)
      }
      frame "Complete" {
        w496 = State."Complete"  # State
        w495 = State."WaitVac"  # State
        w506 = State."Abort"  # State
        # "more_runs?"
        n122 = case shown="True" "Write?" {
          tunnel: w503 -> [_ w521]
          tunnel: [FALSE ("Write_OK") w518] -> w491
          tunnel: [path "" w517] -> w501
          tunnel: "Start_path" -> [_ w516]
          frame False {
          }
          frame True {
            n123 = local read "AI_Start_delay_ms"() -> (w520:dbl)
            n124 = local read "Actual_AI_Rate"() -> (w519:dbl)
            n125 = call "Write_data_to_file.vi"("start_path"=w516, "Start_delay_ms"=w520, "shot_data"=w521, "Actual_AI_Rate"=w519) -> ("Write_OK"=w518:bool, "file_path"=w517:path)  [unwired: 1 in, 1 out]
          }
        }
        "Saved_file_path" <- w501
        "Write_OK" <- w491
        n126 = Less?(x=w486, y=w485) -> (x < y?=w488:bool)
        n127 = And(x=w488, y="Next_run?") -> (x .and. y?=w492:bool)
        n128 = Not(x=w488) -> (.not. x?=w489:bool)
        n129 = And(x=w489, y=w491) -> (x .and. y?=w490:bool)
        n130 = Select(t=w495, s=w492, f=w496) -> (s? t:f=w487:T1)
        n131 = Increment(x=w486) -> (x+1=w493:i32)
        n132 = Or(x=w490, y="Done?") -> (x .or. y?=w500:bool)
        n133 = Select(t=w493, s=w492, f=w486) -> (s? t:f=w494:i32)
        n134 = Select(t=w506, s=w507, f=w487) -> (s? t:f=w505:T1)
      }
      frame "Abort" {
        w532 = State."Abort"  # State
      }
    }
    "6374_data_output" <- w212
    n135 = Select(t=0.0, s=w219, f=2.0) -> (s? t:f=w216:dbl)
    n136 = property on="Write?" class="Bool"("DisabledEnum"=w216) -> ()  [unwired: 2 in, 2 out]
    n137 = Build Array(w180, w179) -> (w210:dbl[])
    n138 = Divide(x=w179, y=w183) -> (x/y=w189:dbl)
    n139 = Divide(x=w180, y=w184) -> (x/y=w186:dbl)
    n140 = property on="Done?" class="Bool"("DisabledEnum"=w216) -> ()  [unwired: 2 in, 2 out]
    n141 = Build Array (concatenate)(w209, w210) -> (w208:dbl[][])
    n142 = Multiply(x=w189, y=100.0) -> (x*y=→"Driver_gauge_%":dbl)
    n143 = Multiply(x=w186, y=100.0) -> (x*y=→"Vac_gauge_%":dbl)
    n144 = Equal?(x=w203, y=w207) -> (x = y?=w202:bool)
    n145 = Equal?(x=w203, y=w206) -> (x = y?=w201:bool)
    n146 = Equal?(x=w203, y=w205) -> (x = y?=w199:bool)
    n147 = Or(x=w202, y=w201) -> (x .or. y?=w200:bool)
    n148 = Or(x=w200, y=w199) -> (x .or. y?=w195:bool)
    n149 = Not(x=w195) -> (.not. x?=→"Vac_Pump":bool)
    n150 = local read "Actual_AI_Rate"() -> (w192:dbl)
    n151 = Build Array(w242, w241) -> (w243:dbl[])
    n152 = call-poly <vilib>:"DAQmx Write.vi"("task/channels in"=w229, "data"=w243, "error in"=w222) -> ("task out"=w244:refnum<k21>, "error out"=w197:errorcluster)  [unwired: 10 in, 1 out]
    n153 = call-poly <vilib>:"DAQmx Write.vi"("task/channels in"=w204, "data"=w195, "error in"=w197) -> ("error out"=w196:errorcluster)  [unwired: 10 in, 2 out]
    n154 = Index Array(array=w212, index (row)=0 ("index")) -> (element=w191:dbl[])  [unwired: 1 in]
    n155 = call "Settling_V_to_Pa.vi"("Actual_AI_Rate"=w192, "V_array"=w191) -> ("P_Pa_array"=→"Settling_chamber_pressure":dbl[])  [unwired: 3 in]
    n156 = Or(x="Force_stop", y=w198) -> (x .or. y?=w214:bool)
    "Iteration" <- w249
    "Current_state" <- w203
    "Run_count" <- w177
  }
  n157 = Build Array(0, 0) -> (w138:i32[])
  n158 = Transpose 2D Array(2D array=w79) -> (transposed array=→"Control_pressures":dbl[][])
  n159 = local read "Fire_AO_Ch"() -> (w63:tag)
  n160 = property on="Control_pressures" class="WFGraph (strict)"("XScale.Multiplier"=0.1 ("X Scale.Offset and Multiplier:Multiplier"), "YScale.Multiplier"=1.0 ("Y Scale.Offset and Multiplier:Multiplier")) -> ()  [unwired: 2 in, 2 out]
  n161 = Build Array(0.0 ("element"), 0.0 ("element")) -> (w60:dbl[])
  n162 = call-poly <vilib>:"DAQmx Write.vi"("task/channels in"=w137, "data"=w138, "error in"=w132) -> ("task out"=w136:refnum<k21>, "error out"=w133:errorcluster)  [unwired: 10 in, 1 out]
  n163 = call <vilib>:"DAQmx Stop Task.vi"("task/channels in"=w136, "error in"=w133) -> ("task out"=w135:refnum<k21>, "error out"=w134:errorcluster)  [unwired: 12 in]
  n164 = call <vilib>:"DAQmx Clear Task.vi"("task in"=w135, "error in"=w134) -> ("error out"=w129:errorcluster)  [unwired: 13 in]
  n165 = call <vilib>:"DAQmx Stop Task.vi"("task/channels in"=w128, "error in"=w129) -> ("task out"=w131:refnum<k21>, "error out"=w130:errorcluster)  [unwired: 12 in]
  n166 = call <vilib>:"DAQmx Clear Task.vi"("task in"=w131, "error in"=w130) -> ("error out"=w95:errorcluster)  [unwired: 13 in]
  n167 = call <vilib>:"DAQmx Stop Task.vi"("task/channels in"=w96, "error in"=w95) -> ("task out"=w98:refnum<k21>, "error out"=w97:errorcluster)  [unwired: 12 in]
  n168 = call <vilib>:"DAQmx Clear Task.vi"("task in"=w98, "error in"=w97) -> ("error out"=w94:errorcluster)  [unwired: 13 in]
  n169 = call <vilib>:"DAQmx Stop Task.vi"("task/channels in"=w54, "error in"=w94) -> ("task out"=w100:refnum<k21>, "error out"=w99:errorcluster)  [unwired: 12 in]
  n170 = call <vilib>:"DAQmx Clear Task.vi"("task in"=w100, "error in"=w99) -> ("error out"=w53:errorcluster)  [unwired: 13 in]
  n171 = call-poly <vilib>:"DAQmx Create Virtual Channel.vi"("physical channels"=w63, "error in"=w53) -> ("task out"=w59:refnum<k21>, "error out"=w58:errorcluster)  [unwired: 12 in]
  n172 = call-poly <vilib>:"DAQmx Write.vi"("task/channels in"=w59, "auto start"=TRUE, "data"=w60, "error in"=w58) -> ("task out"=w57:refnum<k21>, "error out"=w56:errorcluster)  [unwired: 9 in, 1 out]
  n173 = call <vilib>:"DAQmx Clear Task.vi"("task in"=w57, "error in"=w56) -> ("error out"=w52:errorcluster)  [unwired: 13 in]
  n174 = call-poly <vilib>:"DAQmx Write.vi"("task/channels in"=w66, "data"=FALSE, "error in"=w52) -> ("task out"=w67:refnum<k21>, "error out"=w68:errorcluster)  [unwired: 10 in, 1 out]
  n175 = call <vilib>:"DAQmx Stop Task.vi"("task/channels in"=w67, "error in"=w68) -> ("task out"=w72:refnum<k21>, "error out"=w71:errorcluster)  [unwired: 12 in]
  n176 = call <vilib>:"DAQmx Clear Task.vi"("task in"=w72, "error in"=w71) -> ("error out"=w21:errorcluster)  [unwired: 13 in]
  n177 = call <vilib>:"DAQmx Stop Task.vi"("task/channels in"=w14, "error in"=w21) -> ("task out"=w23:refnum<k21>, "error out"=w22:errorcluster)  [unwired: 12 in]
  n178 = call <vilib>:"DAQmx Clear Task.vi"("task in"=w23, "error in"=w22) -> ("error out"=w9:errorcluster)  [unwired: 13 in]
  n179 = call <vilib>:"Clear Errors.vi"("error in (no error)"=w9) -> ("error out"=w17:errorcluster)  [unwired: 5 in, 1 out]
  n180 = call-poly <vilib>:"DAQmx Create Virtual Channel.vi"("lines"=tag "Dev1/port0/line1", "error in"=w17) -> ("task out"=w19:refnum<k21>, "error out"=w18:errorcluster)  [unwired: 12 in]
  n181 = call-poly <vilib>:"DAQmx Write.vi"("task/channels in"=w19, "auto start"=TRUE, "data"=FALSE, "error in"=w18) -> ("task out"=w12:refnum<k21>, "error out"=w11:errorcluster)  [unwired: 9 in, 1 out]
  n182 = call <vilib>:"DAQmx Clear Task.vi"("task in"=w12, "error in"=w11) -> ("error out"=w10:errorcluster)  [unwired: 13 in]
  n183 = Merge Errors(w9, w10) -> (w13:errorcluster)
  n184 = call <vilib>:"Simple Error Handler.vi"("error in (no error)"=w13) -> ()  [unwired: 4 in, 5 out]
